vi "Exit Pulseblaster.vi"(11 "Path to spinapi.dll":path=path "C:/SpinCore/SpinAPI/lib/spinapi64.dll") -> ()   [LabVIEW 2024]
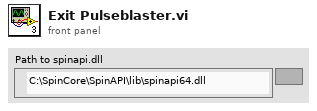
[diagram p1: front panel]
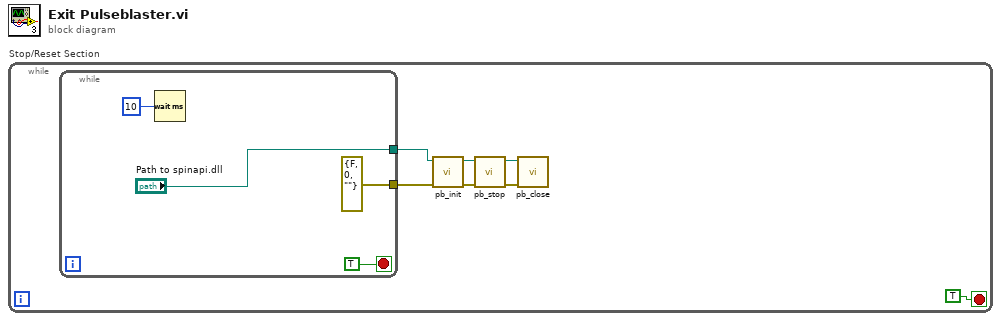
[diagram p0: block diagram]
diagram:
  n1 = while "Stop/Reset Section" {
    stop <- TRUE stop-if-true
    n2 = while {
      tunnel: [errorcluster {"status"=FALSE, "code"=0, "source"=""} ("error in (no error)")] -> w4
      tunnel: ["Path to spinapi.dll"] -> w1
      stop <- TRUE stop-if-true
      n3 = Wait (ms)(milliseconds to wait=u32 10) -> ()  [unwired: 1 out]
    }
    n4 = call "pb_init.vi"("error in (no error)"=w4, "path in"=w1) -> ("error out"=w3:errorcluster, "path out"=w6:path)  [unwired: 1 in, 7 out]
    n5 = call "pb_stop.vi"("error in (no error)"=w3, "path in"=w6) -> ("error out"=w2:errorcluster, "path out"=w7:path)  [unwired: 8 out]
    n6 = call "pb_close.vi"("error in (no error)"=w2, "path in"=w7) -> ()  [unwired: 10 out]
  }
